vi "JSON to Variant.vi"(7 "type in":variant, 8 "error in (no error)":errorcluster, 9 "JSON Data in":variant) -> (0 "error out":errorcluster, 1 "Variant Data out":variant)   [LabVIEW 2019, in "JSON-RPC.lvlib"]
uses:
  JSON-RPC.lvlib
  <vilib>/Utility/Data Type/NI_Data Type.lvlib
  <vilib>/JDP Science/JSONtext/JSONtext.lvlib
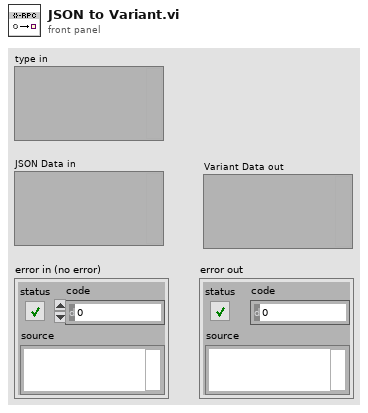
[diagram p1: front panel]
types:
  T1 = typedef "NI_Data Type.lvlib/Data Type.ctl" = enum8{"Invalid Type", "Void", "I8", "I16", "I32", "I64", "U8", "U16", "U32", "U64", "Single Float", "Double Float", "Extended Float", "Single Complex", "Double Complex", "Extended Complex", "Enum U8", "Enum U16", "Enum U32", "Enum U64", "Single Float With Unit", "Double Float With Unit", "Extended Float With Unit", "Single Complex with Unit", "Double Complex with Unit", "Extended Complex with Unit", "Boolean", "String", "Path", "Picture", "Tag", "Array", "Cluster", "Variant", "LV Variant", "Waveform", "Timestamp", "Digital Waveform", "Digital Data", "ExpressData", "Refnum", "External Data", "VI", "Poly VI", "LabVIEW Class Instance", "Fixed Point", "Set Collection", "Map Collection"}
  T2 = typedef "JSONtext.lvlib/JSON Value Type.ctl" = enum16{"Not a JSON Value", "JSON Object", "JSON Array", "String", "Number", "true", "false", "null"}
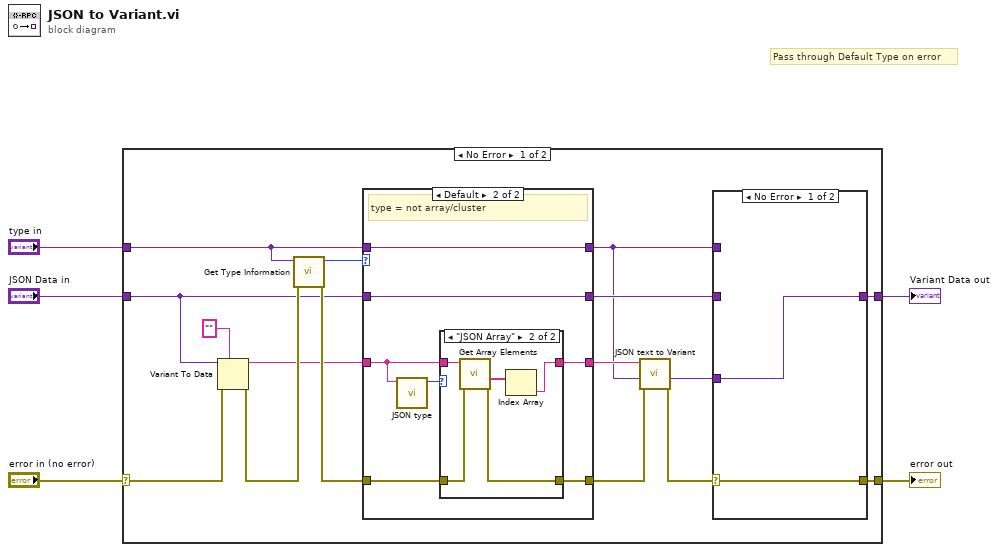
[diagram p0: block diagram]
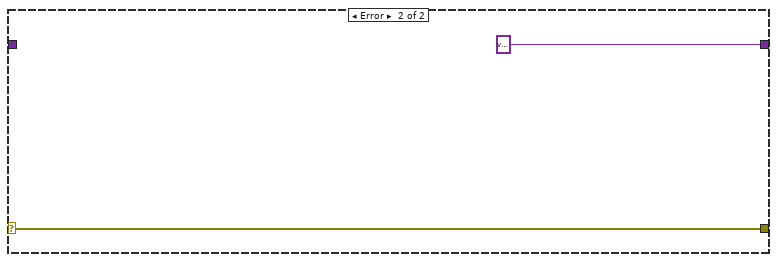
[diagram p5: hidden frame]
diagram:
  # "Pass through Default Type on error"
  n1 = case shown="No Error" "error in (no error)" {
    selector: "error in (no error)" -> [w17 w44]
    tunnel: "JSON Data in" -> [w11 _]
    tunnel: [w12 variant ("Variant")] -> w2
    tunnel: [w15 w44] -> w3
    tunnel: "type in" -> [w19 _]
    frame No Error {
      n2 = Variant To Data(error in=w17, type="", Variant=w11) -> (data=w14:string, error out=w21:errorcluster)
      n3 = call <vilib>:"Get Type Information.vi"("error in (no error)"=w21, "variant"=w19) -> ("error out"=w20:errorcluster, "type"=w16:T1)  [unwired: 5 in, 3 out]
      n4 = case shown="Default" w16 {
        tunnel: [w22 w27] -> w10
        tunnel: [w23 w26] -> w7
        tunnel: w14 -> [w22 w31]
        tunnel: w19 -> [w24 w28]
        tunnel: w20 -> [w23 w29]
        tunnel: [w24 w28] -> w8
        tunnel: [w25 w32] -> w13
        tunnel: w11 -> [w25 w32]
        frame "Array", "Cluster" {
          # "Command = \"\" OR type = Array OR cluster"
        }
        frame Default {
          # "type = not array/cluster"
          n5 = call <vilib>:"JSON type.vi"("JSON"=w31) -> ("JSON Value Type"=w30:T2)  [unwired: 9 in, 1 out]
          n6 = case shown="\"JSON Array\"" w30 {
            tunnel: w31 -> [w33 w38]
            tunnel: [w33 w37] -> w27
            tunnel: w29 -> [w34 w36]
            tunnel: [w34 w35] -> w26
            frame Default {
            }
            frame "JSON Array" {
              n7 = call <vilib>:"Get Array Elements.vi"("error in (no error)"=w36, "JSON"=w38) -> ("error out"=w35:errorcluster, "<JSON>"=w39:string[])  [unwired: 7 in, 1 out]
              n8 = Index Array(array=w39) -> (element=w37:string)  [unwired: 1 in]
            }
          }
        }
      }
      n9 = call <vilib>:"JSON text to Variant.vi"("error in (no error)"=w7, "Data Type"=w8, "JSON"=w10) -> ("error out"=w6:errorcluster, "Variant out"=w9:variant)  [unwired: 7 in]
      n10 = case shown="No Error" w6 {
        selector: w6 -> [w40 _]
        tunnel: [w41 w42] -> w12
        tunnel: w9 -> [w41 _]
        tunnel: [w40 _] -> w15
        tunnel: w13 -> [_ w42]
        tunnel: w8 -> [_ _]
        frame No Error {
        }
        frame Error {
          # "data isn't JSON,\nemit Data in unchanged"
        }
      }
    }
    frame Error {
    }
  }
  "error out" <- w3
  "Variant Data out" <- w2
